vi "OwnCompat20261012_Native_GetTerminalName.vi"() -> ()   [LabVIEW 2024]
panel:
  out "error out":errorcluster caption="错误输出"
  out "terminal_name":string
  in  "terminal_id":u32
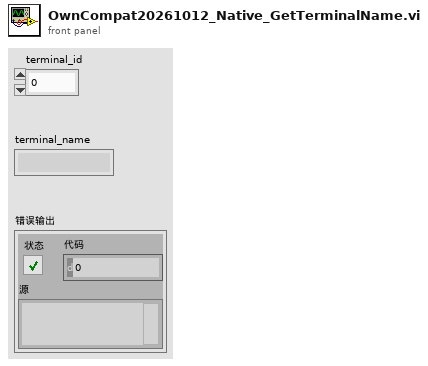
[diagram p1: front panel]
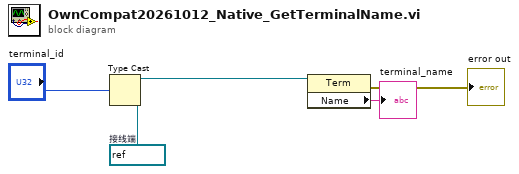
[diagram p0: block diagram]
diagram:
  w4 = refnum<vi> refnum  # 接线端
  n1 = Type Cast ("强制类型转换")(type=w4, x="terminal_id") -> (*(type *) &x=w3:refnum<vi>)
  n2 = property on="属性节点" class="Term"(reference=w3) -> (error out=→"error out":errorcluster, "Name"=→"terminal_name":string)  [unwired: 1 in, 1 out]
